vi "MaP convertir_majuscule.vi"() -> ()   [LabVIEW 2020]
uses:
  LabVIEW-Python TCP Lib/LabVIEW-Python TCP Lib.lvlib
panel:
  out "it":i32
  out "Stop server message":string
  in  "port":u16=5000
  in  "stop":bool
  out "value":T1
  in  "Cluster_de_depart":T2={"fonction"="convertir_majuscule", "parameters"={"chaine"="Et voilà un texte."}}
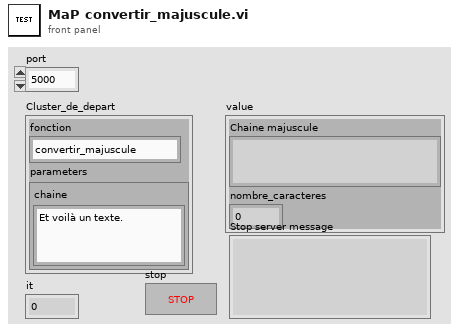
[diagram p1: front panel]
types:
  T1 = cluster{"Chaine majuscule":string, "nombre_caracteres":i32}
  T2 = cluster{"fonction":string, "parameters":cluster{"chaine":string}}
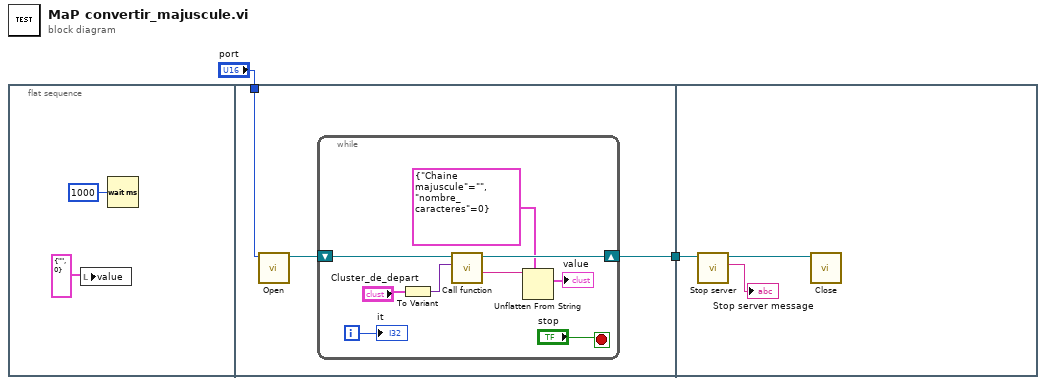
[diagram p0: block diagram]
diagram:
  n1 = flat-sequence {
    tunnel: "port" -> [w6]
    tunnel: [w5] -> w1
    tunnel: w1 -> [w18]
    frame #0 {
      n2 = local write "value"(T1 {"Chaine majuscule"="", "nombre_caracteres"=0} ("value")) -> ()
      n3 = Wait (ms)(milliseconds to wait=u32 1000) -> ()  [unwired: 1 out]
    }
    frame #1 {
      n4 = call "Open.vi"("port"=w6) -> ("connection ID"=w7:refnum<k5>)  [unwired: 9 in, 1 out]
      n5 = while {
        shift-right: [w15] -> w5
        shift-left: w7 -> [w16]
        i -> [w8]
        stop <- "stop" stop-if-true
        n6 = To Variant(anything="Cluster_de_depart") -> (Variant=w11:variant)
        n7 = call "Call function.vi"("variant in"=w11, "connection ID"=w16) -> ("data string out"=w10:string, "connection ID out"=w15:refnum<k5>)  [unwired: 6 in, 2 out]
        n8 = Unflatten From String(type=T1 {"Chaine majuscule"="", "nombre_caracteres"=0}, binary string=w10) -> (value=→"value":T1)  [unwired: 3 in, 2 out]
        "it" <- w8
      }
    }
    frame #2 {
      n9 = call "Stop server.vi"("connection ID"=w18) -> ("Stop server message"=→"Stop server message":string, "connection ID out"=w17:refnum<k5>)  [unwired: 8 in, 1 out]
      n10 = call "Close.vi"("connection ID"=w17) -> ()  [unwired: 9 in, 2 out]
    }
  }
